vi "ReadDIs.vi"(7 "GroveConnector":enum16{"D16", "D18", "D20"}(ring), 8 "error in (no error)":errorcluster, 11 "Session In":refnum<class "Session.lvclass">) -> (0 "error out":errorcluster, 1 "DIStatus 2":bool, 2 "DIStatus 1":bool, 3 "Session Out":refnum<class "Session.lvclass">)   [LabVIEW 2020]
uses:
  CTI/Session/Session.lvclass
  CTI/GPIO Direction.ctl
  CTI/GPIO Number.ctl
  CTI/CTI.lvlib
panel:
  # "Input"
  # "Output"
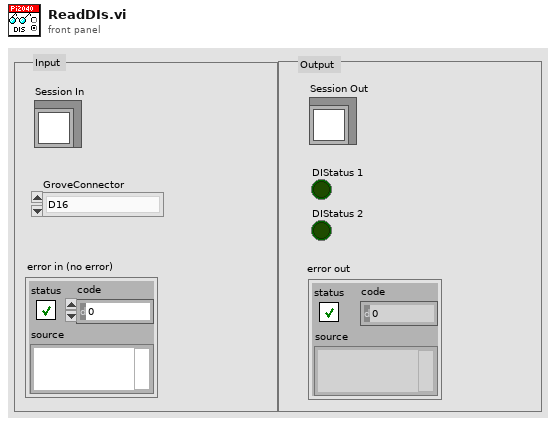
[diagram p1: front panel]
types:
  T1 = typedef "CTI.lvlib/GPIO Direction.ctl" = enum16{"In", "Out"}
  T2 = typedef "CTI.lvlib/GPIO Number.ctl" = i8
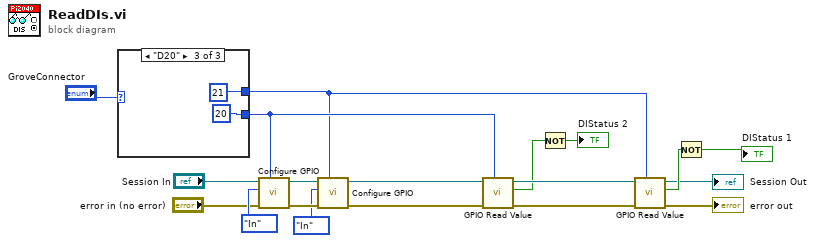
[diagram p0: block diagram]
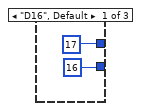
[diagram p2: hidden frame]
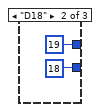
[diagram p3: hidden frame]
diagram:
  n1 = case shown="\"D20\"" "GroveConnector" {
    tunnel: [T2 16 ("GPIO #") T2 18 ("GPIO #") T2 20 ("GPIO #")] -> w5
    tunnel: [T2 17 ("GPIO #") T2 19 ("GPIO #") T2 21 ("GPIO #")] -> w4
    frame "D16", Default {
    }
    frame "D18" {
    }
    frame "D20" {
    }
  }
  n2 = call "Configure GPIO.vi"("GPIO #"=w5, "error in (no error)"="error in (no error)", "GPIO Direction"=GPIO_Direction."In", "Session in"="Session In") -> ("error out"=w18:errorcluster, "Session out"=w17:refnum<class "Session.lvclass">)  [unwired: 6 in]
  n3 = call "Configure GPIO.vi"("GPIO #"=w4, "error in (no error)"=w18, "GPIO Direction"=GPIO_Direction."In", "Session in"=w17) -> ("error out"=w7:errorcluster, "Session out"=w8:refnum<class "Session.lvclass">)  [unwired: 6 in]
  n4 = call "GPIO Read Value.vi"("GPIO #"=w5, "error in (no error)"=w7, "Session in"=w8) -> ("error out"=w14:errorcluster, "Value"=w12:bool, "Session out"=w15:refnum<class "Session.lvclass">)  [unwired: 6 in]
  n5 = Not(x=w12) -> (.not. x?=→"DIStatus 2":bool)
  n6 = call "GPIO Read Value.vi"("GPIO #"=w4, "error in (no error)"=w14, "Session in"=w15) -> ("error out"=→"error out":errorcluster, "Value"=w13:bool, "Session out"=→"Session Out":refnum<class "Session.lvclass">)  [unwired: 6 in]
  n7 = Not(x=w13) -> (.not. x?=→"DIStatus 1":bool)
